vi "Common_UpdateAttributes.vi"(1 "ClassPath/LvClassRef":variant, 2 "NewAttributes":string, 3 "ClassInfo":T4[](array[typedef]), 5 "error in (no error)":errorcluster, 6 "Don't Prompt (False)":bool, 7 "Attributes":T1[](array[typedef]), 8 "Stereotype":string, 9 "Ctl-Description":string) -> (15 "CtlPath":path, 18 "Cancel":bool, 19 "error out":errorcluster)   [LabVIEW 2020] (continued)
                      w703 = 21012 items=[".NET Refnum", "Absolute Value", "Access Rights", "ActiveX Container", "Add", "Add Array Elements", "Agitator", "AllSpoll", "And", "And Array Elements", "Append True/False String", "Application Refnum", "Array", "Array 1", "Array Constant", "Array Max & Min", "Array Size", "Array Subset", "Array To Cluster", "Array To Spreadsheet String", "Array of Strings to Path", "Atmospheric Tank", "Atmospheric Tank 1", "Automation Close", "Automation Open", "Automation Refnum", "Avogadro Constant (1/mol)", "Base 10 Logarithm Of e", "Bin", "Bin 1", "Bluetooth Close Connection", "Bluetooth Create Listener", "Bluetooth Discover", "Bluetooth Network Connection Refnum", "Bluetooth Open Connection", "Bluetooth Read", "Bluetooth Wait On Listener", "Bluetooth Write", "Boolean Array To Number", "Boolean To (0,1)", "Build Array", "Build Cluster Array", "Build Path", "Build Waveform", "Bundle", "Bundle By Name", "Byte Array To String", "Byte Stream File Refnum", "Call By Reference Node", "Call Chain", "Call Library Function Node", "Cancel Button", "Cancel Button 1", "Cancel Notification", "Carriage Return Constant", "Case Structure", "Cast Unit Bases", "Check Valve", "Checkbox", "Class Specifier Constant", "Classic Radio Buttons", "Close File", "Close Reference", "Cluster", "Cluster 1", "Cluster Constant", "Cluster To Array", "Code Interface Node", "Color Box", "Color Box Constant", "Color Box Thin Border", "Color Ramp", "Combo Box", "Combo Box 1", "Combo Box Constant", "Complex Conjugate", "Complex To Polar", "Complex To Re/Im", "Compound Arithmetic", "Compressor", "Concatenate Strings", "Conditional Disable Structure", "Constructor Node", "Control Help Window", "Control Online Help", "Control Refnum", "Convert Unit", "Conveyer", "Copy", "Cosecant", "Cosine", "Cotangent", "Create User Event", "Current VI's Menubar", "Current VI's Path", "DAQmx Analog Trigger Source", "DAQmx Analog Trigger Source 1", "DAQmx Analog Trigger Source 2", "DAQmx Analog Trigger Source Constant", "DAQmx Device Name", "DAQmx Device Name 1", "DAQmx Device Name 2", "DAQmx Device Name Constant", "DAQmx Global Channel", "DAQmx Global Channel 1", "DAQmx Global Channel 2", "DAQmx Global Channel Constant", "DAQmx Physical Channel", "DAQmx Physical Channel 1", "DAQmx Physical Channel 2", "DAQmx Physical Channel Constant", "DAQmx Scale Name", "DAQmx Scale Name 1", "DAQmx Scale Name 2", "DAQmx Scale Name Constant", "DAQmx Switch", "DAQmx Switch 1", "DAQmx Switch 2", "DAQmx Switch Constant", "DAQmx Task Name", "DAQmx Task Name 1", "DAQmx Task Name 2", "DAQmx Task Name Constant", "DAQmx Terminal", "DAQmx Terminal 1", "DAQmx Terminal 2", "DAQmx Terminal Constant", "Data Log File Refnum", "DataSocket Close", "DataSocket Open", "DataSocket Read", "DataSocket Refnum", "DataSocket Write", "Database Variant To Data", "Date/Time To Seconds", "Decimal Digit?", "Decimal String To Number", "Decimate 1D Array", "Decrement", "Default Directory", "Delete", "Delete From Array", "Delete Menu Items", "Delete Variant Attribute", "Delete Waveform Attribute", "Dequeue Element", "Destroy User Event", "DevClear", "DevClearList", "Device Control/Status", "Device Refnum", "Diagram Disable Structure", "Dial", "Dial 1", "Dialog Button", "Dialog Checkbox", "Dialog Chiseled Line", "Dialog Colored Rectangle", "Dialog Combo Box", "Dialog Horizontal Pointer Slide", "Dialog Horizontal Progress Bar", "Dialog Horizontal Slide", "Dialog Label", "Dialog Listbox", "Dialog Listbox 1", "Dialog Multicolumn Listbox", "Dialog Multiple Selection Multicolumn Listbox", "Dialog Numeric", "Dialog Path Control", "Dialog Pict Ring", "Dialog Radio Button", "Dialog Radio Buttons", "Dialog Recessed Frame", "Dialog Ring", "Dialog Spin Control", "Dialog String", "Dialog Tab Control", "Dialog Table", "Dialog Tree", "Dialog Vertical Pointer Slide", "Dialog Vertical Progress Bar", "Dialog Vertical Slide", "Digital Data", "Digital Data 1", "Digital Waveform Graph", "Digital Waveform Graph 1", "Digital Waveform Graph 2", "Divide", "Dlg CheckBox", "Dlg Horiz Scrollbar", "Dlg Numeric", "Dlg Numeric 2", "Dlg String", "Dlg Vert Scrollbar", "Down Arrow", "Down Bow Valve", "Down Bow Valve 1", "Down Bow Valve 2", "Down Rect Valve", "Down Rect Valve 1", "Down Rect Valve 2", "Down Tee", "Down Tee 1", "EOF", "Elementary Charge (C)", "Empty Path Constant", "Empty String Constant", "Empty String/Path?", "Enable Menu Tracking", "EnableLocal", "EnableRemote", "End of Line Constant", "Enqueue Element", "Enqueue Element At Opposite End", "Enum", "Enum 1", "Enum Constant", "Equal To 0?", "Equal?", "Error Ring Constant", "Event Callback Refnum", "Event Structure", "Exchanger", "Exclusive Or", "Exponential", "Exponential (Arg) -1", "Expression Node", "False Constant", "Feedback Node", "FieldPoint IO Point", "FieldPoint IO Point 1", "FieldPoint IO Point Constant", "File Dialog", "File Path Control", "File Path Control 1", "File Path Indicator", "File Path Indicator 1", "File/Directory Info", "FindLstn", "FindRQS", "First Call?", "Flat Box", "Flat Circle", "Flat Down Triangle", "Flat Frame", "Flat Left Triangle", "Flat Right Triangle", "Flat Round Button", "Flat Rounded Box", "Flat Sequence Structure", "Flat Square Button", "Flat Up Triangle", "Flatten To String", "Flatten To XML", "Flattened String To Variant", "Flush File", "Flush Queue", "For Loop", "Format Date/Time String", "Format Into File", "Format Into String", "Format Value", "Formula Node", "Fract/Exp String To Number", "Framed Color Box", "Framed Color Box 1", "Free Label", "Furnace", "GPIB Clear", "GPIB Initialization", "GPIB Misc", "GPIB Read", "GPIB Serial Poll", "GPIB Status", "GPIB Trigger", "GPIB Wait", "GPIB Write", "Gauge", "Gauge 1", "Generate Front Panel Activity", "Generate Occurrence", "Generate User Event", "Generic Refnum", "Generic Refnum By Reference Flatten", "Generic Refnum Deep Copy", "Generic Refnum Name", "Generic Refnum Tag", "Generic Refnum Tag By Reference Flatten", "Generic Refnum Tag Flatten", "Get Date/Time In Seconds", "Get Date/Time String", "Get Help Window Status", "Get Menu Item Info", "Get Menu Selection", "Get Menu Short Cut Info", "Get Notifier Status", "Get Queue Status", "Get Variant Attribute", "Get Waveform Attribute", "Get Waveform Components", "Global Variable", "Gravitational Constant (N m2/kg2)", "Greater Or Equal To 0?", "Greater Or Equal?", "Greater Than 0?", "Greater?", "Handle Peek", "Handle Poke", "Hex Digit?", "Hexadecimal String To Number", "HiQ-Script", "Hopper", "Hopper 1", "Horiz Line", "Horiz Pipe", "Horiz Pipe 1", "Horizontal Button Box", "Horizontal Fill Slide", "Horizontal Fill Slide 1", "Horizontal Graduated Bar", "Horizontal Pointer Slide", "Horizontal Pointer Slide 1", "Horizontal Progress Bar", "Horizontal Slide", "Horizontal Slide Switch", "Horizontal Smooth Box", "Horizontal Switch", "Horizontal Tank", "Horizontal Toggle Switch", "Horizontal Toggle Switch 1", "Hyperbolic Cosine", "Hyperbolic Sine", "Hyperbolic Tangent", "IMAQ Session", "IP To String", "IVI Delete Session", "IVI Logical Name", "IVI Logical Name 1", "IVI Logical Name Constant", "IVI New Session", "Implies", "In Range and Coerce", "Increment", "Index & Bundle Cluster Array", "Index Array", "Index String Array", "Initialize Array", "Insert Into Array", "Insert Menu Items", "Intensity Chart", "Intensity Chart 1", "Intensity Graph", "Intensity Graph 1", "Interleave 1D Arrays", "Interpolate 1D Array", "Inverse Cosine", "Inverse Hyperbolic Cosine", "Inverse Hyperbolic Sine", "Inverse Hyperbolic Tangent", "Inverse Sine", "Inverse Tangent", "Inverse Tangent (2 Input)", "Invoke Node", "IrDA Close Connection", "IrDA Create Listener", "IrDA Discover", "IrDA Network Connection Refnum", "IrDA Open Connection", "IrDA Read", "IrDA Wait On Listener", "IrDA Write", "Join Numbers", "Knob", "Knob 1", "LED Button", "Label", "Labeled Oblong Button", "Labeled Rectangular Button", "Labeled Round Button", "Labeled Square Button", "Left Arrow", "Left Bow Valve", "Left Bow Valve 1", "Left Bow Valve 2", "Left Down Elbow", "Left Down Elbow 1", "Left Pump", "Left Pump 1", "Left Rect Valve", "Left Rect Valve 1", "Left Rect Valve 2", "Left Tee", "Left Tee 1", "Left Up Elbow", "Left Up Elbow 1", "Less Or Equal To 0?", "Less Or Equal?", "Less Than 0?", "Less?", "Lexical Class", "Line Feed Constant", "List Directory", "Listbox", "Listbox 1", "Listbox Symbol Ring Constant", "Local Variable", "Lock Range", "Logarithm Base 10", "Logarithm Base 2", "Logarithm Base X", "Logical Shift", "Lowered Rounded Box", "MATLAB Script", "MakeAddr", "Mantissa & Exponent", "Match First String", "Match Pattern", "Match True/False String", "Max & Min", "Menu Refnum", "Menu Ring", "Menu Ring 1", "Menu-Popup Ring", "Merge Signals", "Meter", "Meter 1", "Molar Gas Constant (J/(mol K))", "Motion Resource", "Motion Resource 1", "Motion Resource Constant", "Motor", "Motor 1", "Move", "Multicolumn Listbox", "Multicolumn Listbox 1", "Multicolumn Listbox 2", "Multicolumn Listbox 3", "Multicolumn Listbox 4", "Multiple Selection Listbox", "Multiple Selection Listbox 1", "Multiple Selection Listbox 2", "Multiple Selection Listbox 3", "Multiple Selection Multicolumn Listbox", "Multiply", "Multiply Array Elements", "Natural Logarithm", "Natural Logarithm (Arg +1)", "Natural Logarithm Base", "Natural Logarithm Of 10", "Natural Logarithm Of 2", "Natural Logarithm Of Pi", "Negate", "Negative Infinity", "New Directory", "New File", "New VI", "New VI Object", "Not", "Not A Number/Path/Refnum?", "Not A Path Constant", "Not And", "Not Equal To 0?", "Not Equal?", "Not Exclusive Or", "Not Or", "Not a Refnum Constant", "Not a Tag", "Number To Boolean Array", "Number To Decimal String", "Number To Engineering String", "Number To Exponential String", "Number To Fractional String", "Number To Hexadecimal String", "Number To Octal String", "Numeric Constant", "Numeric Control", "Numeric Control 1", "Numeric Indicator", "Numeric Indicator 1", "OK Button", "OLE Variant", "Obtain Notifier", "Obtain Queue", "Occurrence Refnum", "Octal Digit?", "Octal String To Number", "Old VISA Open", "One Button Dialog", "Open Application Reference", "Open Device", "Open File", "Open File (New)", "Open Tank", "Open Tank 1", "Open VI Object Reference", "Open VI Reference", "Or", "Or Array Elements", "PPoll", "PPollConfig", "PPollUnconfig", "PassControl", "Path Constant", "Path To String", "Path Type", "Path to Array of Strings", "Pi", "Pi Divided By 2", "Pi Multiplied By 2", "Pick Line", "Pict Ring", "Pict Ring 1", "Picture", "PixMap", "PixMap (Do not touch it!!)", "Planck Constant (J/Hz)", "Platform Flat Square Button", "Plug-In Control", "Polar To Complex", "Positive Infinity", "Power Of 10", "Power Of 2", "Power Of X", "Pressure Tank", "Pressure Tank 1", "Preview Queue Element", "Printable?", "Property Node", "Pulldown Menu Ring", "Push Button", "Quit LabVIEW", "Quotient & Remainder", "Radio Buttons", "Raised Box", "Raised Box 1", "Raised Circle", "Raised Down Triangle", "Raised Frame", "Raised Left Triangle", "Raised Right Triangle", "Raised Rounded Box", "Raised Up Triangle", "Random Number (0-1)", "RcvRespMsg", "Re/Im To Complex", "Read Binary File", "Read Device", "Read File", "ReadStatus", "Receive", "ReceiveSetup", "Recessed Box", "Recessed Circle", "Recessed Down Triangle", "Recessed Frame", "Recessed Left Triangle", "Recessed Menu Ring", "Recessed Right Triangle", "Recessed Rounded Box", "Recessed Up Triangle", "Reciprocal", "Reciprocal Of Pi", "Reciprocal Of e", "Rectangular Stop Button", "Refnum to Path", "Refnum to Session", "Register Event Callback", "Register For Events", "Register Session", "Release Notifier", "Release Queue", "Replace Array Subset", "Replace Substring", "Request Deallocation", "ResetSys", "Reshape Array", "Reverse 1D Array", "Reverse String", "Right Arrow", "Right Bow Valve", "Right Bow Valve 1", "Right Bow Valve 2", "Right Down Elbow", "Right Down Elbow 1", "Right Pump", "Right Pump 1", "Right Rect Valve", "Right Rect Valve 1", "Right Rect Valve 2", "Right Tee", "Right Tee 1", "Right Up Elbow", "Right Up Elbow 1", "Ring Constant", "Rocker", "Rotary Feeder", "Rotate", "Rotate 1D Array", "Rotate Left With Carry", "Rotate Right With Carry", "Rotate String", "Round Button", "Round LED", "Round LED 1", "Round Light", "Round Push Button", "Round Push Button 2", "Round Radio Button", "Round Stop Button", "Round To +Infinity", "Round To -Infinity", "Round To Nearest", "Rydberg Constant (/m)", "Scale By Power Of 2", "Scan From File", "Scan From String", "Scan String For Tokens", "Scan Value", "Search 1D Array", "Search and Replace String", "Search/Split String", "Secant", "Seconds To Date/Time", "Seek", "Select", "Send", "Send Notification", "SendCmds", "SendDataBytes", "SendIFC", "SendLLO", "SendList", "SendSetup", "Session to Refnum", "Set Menu Item Info", "Set Occurrence", "Set Variant Attribute", "Set Waveform Attribute", "SetRWLS", "SetTimeOut", "Sign", "Simple Horizontal Slide", "Simple Numeric", "Simple Numeric 1", "Simple String", "Simple Vertical Slide", "Simulation Loop", "Sinc", "Sine", "Sine & Cosine", "Single Selection Listbox", "Size Handle", "Slide Switch", "Sort 1D Array", "Speed Of Light In Vacuum (m/sec)", "Split 1D Array", "Split Button", "Split Number", "Split Signals", "Spreadsheet String To Array", "Square Button", "Square LED", "Square LED 1", "Square Light", "Square Push Button", "Square Push Button 2", "Square Radio Button", "Square Root", "Stacked Sequence Structure", "Standard ListBox", "State Diagram", "Static VI Reference", "Stop", "Stop Button", "String Constant", "String Control", "String Control 1", "String Indicator", "String Indicator 1", "String Length", "String Subset", "String To Byte Array", "String To IP", "String To Path", "String to Tag", "Strip Path", "SubPanel", "SubPanel (Classic)", "Subtract", "Swap Bytes", "Swap Vector Element", "Swap Words", "TCP Close Connection", "TCP Create Listener", "TCP Flattened Read", "TCP Flattened Write", "TCP Flex Read", "TCP Flex Write", "TCP Network Connection Refnum", "TCP Open Connection", "TCP Read", "TCP Wait On Listener", "TCP Write", "Tab Constant", "Tab Control", "Tab Control 1", "Table", "Table 1", "Table 2", "Tag Attribute Ring", "Tag Constant", "Tag Control", "Tag Control 1", "Tag Indicator", "Tag Indicator 1", "Tag to String", "Tangent", "Tank", "Tank 1", "Temporary Directory", "TestSRQ", "TestSys", "Text & Pict Ring", "Text & Pict Ring 1", "Text Button", "Text Ring", "Text Ring 1", "Thermometer", "Thermometer 1", "Thick Chiseled Line", "Thick Line", "Thick Line with Arrow", "Thick Lowered Box", "Thin Chiseled Line", "Thin Line", "Thin Line with Arrow", "Threshold 1D Array", "Tick Count (ms)", "Time Stamp Constant", "Time Stamp Control", "Time Stamp Control 1", "Time Stamp Indicator", "Time Stamp Indicator 1", "Timed Loop", "To Byte Integer", "To Double Precision Complex", "To Double Precision Float", "To Extended Precision Complex", "To Extended Precision Float", "To Long Integer", "To Lower Case", "To More Generic Class", "To More Specific Class", "To OLE Variant", "To Quad Integer", "To Single Precision Complex", "To Single Precision Float", "To Time Stamp", "To Unsigned Byte Integer", "To Unsigned Long Integer", "To Unsigned Quad Integer", "To Unsigned Word Integer", "To Upper Case", "To Variant", "To Word Integer", "Traditional DAQ Channel", "Traditional DAQ Channel 1", "Traditional DAQ Channel Constant", "Transpose 2D Array", "Tree", "Trigger", "TriggerList", "Two Button Dialog", "Type Cast", "Type and Creator", "UDP Close", "UDP Multicast Open", "UDP Network Connection Refnum", "UDP Open", "UDP Read", "UDP Write", "Unbundle", "Unbundle By Name", "Unflatten From String", "Unflatten From XML", "Uniform Dbl Waveform", "Uniform Int16 Waveform", "Unregister For Events", "Unregister Session", "Up Arrow", "Up Bow Valve", "Up Bow Valve 1", "Up Bow Valve 2", "Up Rect Valve", "Up Rect Valve 1", "Up Rect Valve 2", "Up Tee", "Up Tee 1", "User Item", "VI Library", "VI Refnum", "VISA Assert Interrupt Signal", "VISA Assert Trigger", "VISA Assert Utility Signal", "VISA Clear", "VISA Close", "VISA Disable Event", "VISA Discard Events", "VISA Enable Event", "VISA Find Resource", "VISA Flush I/O Buffer", "VISA GPIB Command", "VISA GPIB Control ATN", "VISA GPIB Control REN", "VISA GPIB Pass Control", "VISA GPIB Send IFC", "VISA In 16", "VISA In 32", "VISA In 8", "VISA Lock", "VISA Map Address", "VISA Map Trigger", "VISA Memory Allocation", "VISA Memory Free", "VISA Move", "VISA Move In 16", "VISA Move In 32", "VISA Move In 8", "VISA Move Out 16", "VISA Move Out 32", "VISA Move Out 8", "VISA Open", "VISA Out 16", "VISA Out 32", "VISA Out 8", "VISA Peek 16", "VISA Peek 32", "VISA Peek 8", "VISA Poke 16", "VISA Poke 32", "VISA Poke 8", "VISA Read", "VISA Read STB", "VISA Read To File", "VISA Refnum to Session", "VISA Resource Name", "VISA Resource Name Constant", "VISA Set I/O Buffer Size", "VISA Status Description", "VISA USB Control In", "VISA USB Control Out", "VISA Unlock", "VISA Unmap Address", "VISA Unmap Trigger", "VISA VXI Cmd or Query", "VISA Wait on Event", "VISA Write", "VISA Write From File", "VISA resource name", "Variant", "Variant To Data", "Variant To Flattened String", "Vert Line", "Vert Pipe", "Vert Pipe 1", "Vert Rocker", "Vertical Fill Slide", "Vertical Fill Slide 1", "Vertical Graduated Bar", "Vertical Pointer Slide", "Vertical Pointer Slide 1", "Vertical Progress Bar", "Vertical Slide", "Vertical Slide Switch", "Vertical Slide Switch 1", "Vertical Smooth Box", "Vertical Switch", "Vertical Toggle Switch", "Vertical Toggle Switch 1", "Volume Info", "Wait (ms)", "Wait For Activity", "Wait For Front Panel Activity", "Wait Until Next ms Multiple", "Wait for GPIB RQS", "Wait on Notification", "Wait on Notification from Multiple", "Wait on Occurrence", "WaitSRQ", "Waveform Chart", "Waveform Chart 1", "Waveform Chart 2", "Waveform Graph", "Waveform Graph 1", "While Loop", "While Loop 1", "White Space?", "Write Device", "Write File", "XY Graph", "XY Graph 1", "Xmath Script"]
                      w706 = refnum<vi> refnum  # Cluster
                      w707 = 3400 items=[".NET Refnum", "Absolute Value", "Access Rights", "ActiveX Container", "Add", "Add Array Elements", "Agitator", "AllSpoll", "And", "And Array Elements", "Append True/False String", "Application Refnum", "Array", "Array 1", "Array Constant", "Array Max & Min", "Array Size", "Array Subset", "Array To Cluster", "Array To Spreadsheet String", "Array of Strings to Path", "Atmospheric Tank", "Atmospheric Tank 1", "Automation Close", "Automation Open", "Automation Refnum", "Avogadro Constant (1/mol)", "Base 10 Logarithm Of e", "Bin", "Bin 1", "Bluetooth Close Connection", "Bluetooth Create Listener", "Bluetooth Discover", "Bluetooth Network Connection Refnum", "Bluetooth Open Connection", "Bluetooth Read", "Bluetooth Wait On Listener", "Bluetooth Write", "Boolean Array To Number", "Boolean To (0,1)", "Build Array", "Build Cluster Array", "Build Path", "Build Waveform", "Bundle", "Bundle By Name", "Byte Array To String", "Byte Stream File Refnum", "Call By Reference Node", "Call Chain", "Call Library Function Node", "Cancel Button", "Cancel Button 1", "Cancel Notification", "Carriage Return Constant", "Case Structure", "Cast Unit Bases", "Check Valve", "Checkbox", "Class Specifier Constant", "Classic Radio Buttons", "Close File", "Close Reference", "Cluster", "Cluster 1", "Cluster Constant", "Cluster To Array", "Code Interface Node", "Color Box", "Color Box Constant", "Color Box Thin Border", "Color Ramp", "Combo Box", "Combo Box 1", "Combo Box Constant", "Complex Conjugate", "Complex To Polar", "Complex To Re/Im", "Compound Arithmetic", "Compressor", "Concatenate Strings", "Conditional Disable Structure", "Constructor Node", "Control Help Window", "Control Online Help", "Control Refnum", "Convert Unit", "Conveyer", "Copy", "Cosecant", "Cosine", "Cotangent", "Create User Event", "Current VI's Menubar", "Current VI's Path", "DAQmx Analog Trigger Source", "DAQmx Analog Trigger Source 1", "DAQmx Analog Trigger Source 2", "DAQmx Analog Trigger Source Constant", "DAQmx Device Name", "DAQmx Device Name 1", "DAQmx Device Name 2", "DAQmx Device Name Constant", "DAQmx Global Channel", "DAQmx Global Channel 1", "DAQmx Global Channel 2", "DAQmx Global Channel Constant", "DAQmx Physical Channel", "DAQmx Physical Channel 1", "DAQmx Physical Channel 2", "DAQmx Physical Channel Constant", "DAQmx Scale Name", "DAQmx Scale Name 1", "DAQmx Scale Name 2", "DAQmx Scale Name Constant", "DAQmx Switch", "DAQmx Switch 1", "DAQmx Switch 2", "DAQmx Switch Constant", "DAQmx Task Name", "DAQmx Task Name 1", "DAQmx Task Name 2", "DAQmx Task Name Constant", "DAQmx Terminal", "DAQmx Terminal 1", "DAQmx Terminal 2", "DAQmx Terminal Constant", "Data Log File Refnum", "DataSocket Close", "DataSocket Open", "DataSocket Read", "DataSocket Refnum", "DataSocket Write", "Database Variant To Data", "Date/Time To Seconds", "Decimal Digit?", "Decimal String To Number", "Decimate 1D Array", "Decrement", "Default Directory", "Delete", "Delete From Array", "Delete Menu Items", "Delete Variant Attribute", "Delete Waveform Attribute", "Dequeue Element", "Destroy User Event", "DevClear", "DevClearList", "Device Control/Status", "Device Refnum", "Diagram Disable Structure", "Dial", "Dial 1", "Dialog Button", "Dialog Checkbox", "Dialog Chiseled Line", "Dialog Colored Rectangle", "Dialog Combo Box", "Dialog Horizontal Pointer Slide", "Dialog Horizontal Progress Bar", "Dialog Horizontal Slide", "Dialog Label", "Dialog Listbox", "Dialog Listbox 1", "Dialog Multicolumn Listbox", "Dialog Multiple Selection Multicolumn Listbox", "Dialog Numeric", "Dialog Path Control", "Dialog Pict Ring", "Dialog Radio Button", "Dialog Radio Buttons", "Dialog Recessed Frame", "Dialog Ring", "Dialog Spin Control", "Dialog String", "Dialog Tab Control", "Dialog Table", "Dialog Tree", "Dialog Vertical Pointer Slide", "Dialog Vertical Progress Bar", "Dialog Vertical Slide", "Digital Data", "Digital Data 1", "Digital Waveform Graph", "Digital Waveform Graph 1", "Digital Waveform Graph 2", "Divide", "Dlg CheckBox", "Dlg Horiz Scrollbar", "Dlg Numeric", "Dlg Numeric 2", "Dlg String", "Dlg Vert Scrollbar", "Down Arrow", "Down Bow Valve", "Down Bow Valve 1", "Down Bow Valve 2", "Down Rect Valve", "Down Rect Valve 1", "Down Rect Valve 2", "Down Tee", "Down Tee 1", "EOF", "Elementary Charge (C)", "Empty Path Constant", "Empty String Constant", "Empty String/Path?", "Enable Menu Tracking", "EnableLocal", "EnableRemote", "End of Line Constant", "Enqueue Element", "Enqueue Element At Opposite End", "Enum", "Enum 1", "Enum Constant", "Equal To 0?", "Equal?", "Error Ring Constant", "Event Callback Refnum", "Event Structure", "Exchanger", "Exclusive Or", "Exponential", "Exponential (Arg) -1", "Expression Node", "False Constant", "Feedback Node", "FieldPoint IO Point", "FieldPoint IO Point 1", "FieldPoint IO Point Constant", "File Dialog", "File Path Control", "File Path Control 1", "File Path Indicator", "File Path Indicator 1", "File/Directory Info", "FindLstn", "FindRQS", "First Call?", "Flat Box", "Flat Circle", "Flat Down Triangle", "Flat Frame", "Flat Left Triangle", "Flat Right Triangle", "Flat Round Button", "Flat Rounded Box", "Flat Sequence Structure", "Flat Square Button", "Flat Up Triangle", "Flatten To String", "Flatten To XML", "Flattened String To Variant", "Flush File", "Flush Queue", "For Loop", "Format Date/Time String", "Format Into File", "Format Into String", "Format Value", "Formula Node", "Fract/Exp String To Number", "Framed Color Box", "Framed Color Box 1", "Free Label", "Furnace", "GPIB Clear", "GPIB Initialization", "GPIB Misc", "GPIB Read", "GPIB Serial Poll", "GPIB Status", "GPIB Trigger", "GPIB Wait", "GPIB Write", "Gauge", "Gauge 1", "Generate Front Panel Activity", "Generate Occurrence", "Generate User Event", "Generic Refnum", "Generic Refnum By Reference Flatten", "Generic Refnum Deep Copy", "Generic Refnum Name", "Generic Refnum Tag", "Generic Refnum Tag By Reference Flatten", "Generic Refnum Tag Flatten", "Get Date/Time In Seconds", "Get Date/Time String", "Get Help Window Status", "Get Menu Item Info", "Get Menu Selection", "Get Menu Short Cut Info", "Get Notifier Status", "Get Queue Status", "Get Variant Attribute", "Get Waveform Attribute", "Get Waveform Components", "Global Variable", "Gravitational Constant (N m2/kg2)", "Greater Or Equal To 0?", "Greater Or Equal?", "Greater Than 0?", "Greater?", "Handle Peek", "Handle Poke", "Hex Digit?", "Hexadecimal String To Number", "HiQ-Script", "Hopper", "Hopper 1", "Horiz Line", "Horiz Pipe", "Horiz Pipe 1", "Horizontal Button Box", "Horizontal Fill Slide", "Horizontal Fill Slide 1", "Horizontal Graduated Bar", "Horizontal Pointer Slide", "Horizontal Pointer Slide 1", "Horizontal Progress Bar", "Horizontal Slide", "Horizontal Slide Switch", "Horizontal Smooth Box", "Horizontal Switch", "Horizontal Tank", "Horizontal Toggle Switch", "Horizontal Toggle Switch 1", "Hyperbolic Cosine", "Hyperbolic Sine", "Hyperbolic Tangent", "IMAQ Session", "IP To String", "IVI Delete Session", "IVI Logical Name", "IVI Logical Name 1", "IVI Logical Name Constant", "IVI New Session", "Implies", "In Range and Coerce", "Increment", "Index & Bundle Cluster Array", "Index Array", "Index String Array", "Initialize Array", "Insert Into Array", "Insert Menu Items", "Intensity Chart", "Intensity Chart 1", "Intensity Graph", "Intensity Graph 1", "Interleave 1D Arrays", "Interpolate 1D Array", "Inverse Cosine", "Inverse Hyperbolic Cosine", "Inverse Hyperbolic Sine", "Inverse Hyperbolic Tangent", "Inverse Sine", "Inverse Tangent", "Inverse Tangent (2 Input)", "Invoke Node", "IrDA Close Connection", "IrDA Create Listener", "IrDA Discover", "IrDA Network Connection Refnum", "IrDA Open Connection", "IrDA Read", "IrDA Wait On Listener", "IrDA Write", "Join Numbers", "Knob", "Knob 1", "LED Button", "Label", "Labeled Oblong Button", "Labeled Rectangular Button", "Labeled Round Button", "Labeled Square Button", "Left Arrow", "Left Bow Valve", "Left Bow Valve 1", "Left Bow Valve 2", "Left Down Elbow", "Left Down Elbow 1", "Left Pump", "Left Pump 1", "Left Rect Valve", "Left Rect Valve 1", "Left Rect Valve 2", "Left Tee", "Left Tee 1", "Left Up Elbow", "Left Up Elbow 1", "Less Or Equal To 0?", "Less Or Equal?", "Less Than 0?", "Less?", "Lexical Class", "Line Feed Constant", "List Directory", "Listbox", "Listbox 1", "Listbox Symbol Ring Constant", "Local Variable", "Lock Range", "Logarithm Base 10", "Logarithm Base 2", "Logarithm Base X", "Logical Shift", "Lowered Rounded Box", "MATLAB Script", "MakeAddr", "Mantissa & Exponent", "Match First String", "Match Pattern", "Match True/False String", "Max & Min", "Menu Refnum", "Menu Ring", "Menu Ring 1", "Menu-Popup Ring", "Merge Signals", "Meter", "Meter 1", "Molar Gas Constant (J/(mol K))", "Motion Resource", "Motion Resource 1", "Motion Resource Constant", "Motor", "Motor 1", "Move", "Multicolumn Listbox", "Multicolumn Listbox 1", "Multicolumn Listbox 2", "Multicolumn Listbox 3", "Multicolumn Listbox 4", "Multiple Selection Listbox", "Multiple Selection Listbox 1", "Multiple Selection Listbox 2", "Multiple Selection Listbox 3", "Multiple Selection Multicolumn Listbox", "Multiply", "Multiply Array Elements", "Natural Logarithm", "Natural Logarithm (Arg +1)", "Natural Logarithm Base", "Natural Logarithm Of 10", "Natural Logarithm Of 2", "Natural Logarithm Of Pi", "Negate", "Negative Infinity", "New Directory", "New File", "New VI", "New VI Object", "Not", "Not A Number/Path/Refnum?", "Not A Path Constant", "Not And", "Not Equal To 0?", "Not Equal?", "Not Exclusive Or", "Not Or", "Not a Refnum Constant", "Not a Tag", "Number To Boolean Array", "Number To Decimal String", "Number To Engineering String", "Number To Exponential String", "Number To Fractional String", "Number To Hexadecimal String", "Number To Octal String", "Numeric Constant", "Numeric Control", "Numeric Control 1", "Numeric Indicator", "Numeric Indicator 1", "OK Button", "OLE Variant", "Obtain Notifier", "Obtain Queue", "Occurrence Refnum", "Octal Digit?", "Octal String To Number", "Old VISA Open", "One Button Dialog", "Open Application Reference", "Open Device", "Open File", "Open File (New)", "Open Tank", "Open Tank 1", "Open VI Object Reference", "Open VI Reference", "Or", "Or Array Elements", "PPoll", "PPollConfig", "PPollUnconfig", "PassControl", "Path Constant", "Path To String", "Path Type", "Path to Array of Strings", "Pi", "Pi Divided By 2", "Pi Multiplied By 2", "Pick Line", "Pict Ring", "Pict Ring 1", "Picture", "PixMap", "PixMap (Do not touch it!!)", "Planck Constant (J/Hz)", "Platform Flat Square Button", "Plug-In Control", "Polar To Complex", "Positive Infinity", "Power Of 10", "Power Of 2", "Power Of X", "Pressure Tank", "Pressure Tank 1", "Preview Queue Element", "Printable?", "Property Node", "Pulldown Menu Ring", "Push Button", "Quit LabVIEW", "Quotient & Remainder", "Radio Buttons", "Raised Box", "Raised Box 1", "Raised Circle", "Raised Down Triangle", "Raised Frame", "Raised Left Triangle", "Raised Right Triangle", "Raised Rounded Box", "Raised Up Triangle", "Random Number (0-1)", "RcvRespMsg", "Re/Im To Complex", "Read Binary File", "Read Device", "Read File", "ReadStatus", "Receive", "ReceiveSetup", "Recessed Box", "Recessed Circle", "Recessed Down Triangle", "Recessed Frame", "Recessed Left Triangle", "Recessed Menu Ring", "Recessed Right Triangle", "Recessed Rounded Box", "Recessed Up Triangle", "Reciprocal", "Reciprocal Of Pi", "Reciprocal Of e", "Rectangular Stop Button", "Refnum to Path", "Refnum to Session", "Register Event Callback", "Register For Events", "Register Session", "Release Notifier", "Release Queue", "Replace Array Subset", "Replace Substring", "Request Deallocation", "ResetSys", "Reshape Array", "Reverse 1D Array", "Reverse String", "Right Arrow", "Right Bow Valve", "Right Bow Valve 1", "Right Bow Valve 2", "Right Down Elbow", "Right Down Elbow 1", "Right Pump", "Right Pump 1", "Right Rect Valve", "Right Rect Valve 1", "Right Rect Valve 2", "Right Tee", "Right Tee 1", "Right Up Elbow", "Right Up Elbow 1", "Ring Constant", "Rocker", "Rotary Feeder", "Rotate", "Rotate 1D Array", "Rotate Left With Carry", "Rotate Right With Carry", "Rotate String", "Round Button", "Round LED", "Round LED 1", "Round Light", "Round Push Button", "Round Push Button 2", "Round Radio Button", "Round Stop Button", "Round To +Infinity", "Round To -Infinity", "Round To Nearest", "Rydberg Constant (/m)", "Scale By Power Of 2", "Scan From File", "Scan From String", "Scan String For Tokens", "Scan Value", "Search 1D Array", "Search and Replace String", "Search/Split String", "Secant", "Seconds To Date/Time", "Seek", "Select", "Send", "Send Notification", "SendCmds", "SendDataBytes", "SendIFC", "SendLLO", "SendList", "SendSetup", "Session to Refnum", "Set Menu Item Info", "Set Occurrence", "Set Variant Attribute", "Set Waveform Attribute", "SetRWLS", "SetTimeOut", "Sign", "Simple Horizontal Slide", "Simple Numeric", "Simple Numeric 1", "Simple String", "Simple Vertical Slide", "Simulation Loop", "Sinc", "Sine", "Sine & Cosine", "Single Selection Listbox", "Size Handle", "Slide Switch", "Sort 1D Array", "Speed Of Light In Vacuum (m/sec)", "Split 1D Array", "Split Button", "Split Number", "Split Signals", "Spreadsheet String To Array", "Square Button", "Square LED", "Square LED 1", "Square Light", "Square Push Button", "Square Push Button 2", "Square Radio Button", "Square Root", "Stacked Sequence Structure", "Standard ListBox", "State Diagram", "Static VI Reference", "Stop", "Stop Button", "String Constant", "String Control", "String Control 1", "String Indicator", "String Indicator 1", "String Length", "String Subset", "String To Byte Array", "String To IP", "String To Path", "String to Tag", "Strip Path", "SubPanel", "SubPanel (Classic)", "Subtract", "Swap Bytes", "Swap Vector Element", "Swap Words", "TCP Close Connection", "TCP Create Listener", "TCP Flattened Read", "TCP Flattened Write", "TCP Flex Read", "TCP Flex Write", "TCP Network Connection Refnum", "TCP Open Connection", "TCP Read", "TCP Wait On Listener", "TCP Write", "Tab Constant", "Tab Control", "Tab Control 1", "Table", "Table 1", "Table 2", "Tag Attribute Ring", "Tag Constant", "Tag Control", "Tag Control 1", "Tag Indicator", "Tag Indicator 1", "Tag to String", "Tangent", "Tank", "Tank 1", "Temporary Directory", "TestSRQ", "TestSys", "Text & Pict Ring", "Text & Pict Ring 1", "Text Button", "Text Ring", "Text Ring 1", "Thermometer", "Thermometer 1", "Thick Chiseled Line", "Thick Line", "Thick Line with Arrow", "Thick Lowered Box", "Thin Chiseled Line", "Thin Line", "Thin Line with Arrow", "Threshold 1D Array", "Tick Count (ms)", "Time Stamp Constant", "Time Stamp Control", "Time Stamp Control 1", "Time Stamp Indicator", "Time Stamp Indicator 1", "Timed Loop", "To Byte Integer", "To Double Precision Complex", "To Double Precision Float", "To Extended Precision Complex", "To Extended Precision Float", "To Long Integer", "To Lower Case", "To More Generic Class", "To More Specific Class", "To OLE Variant", "To Quad Integer", "To Single Precision Complex", "To Single Precision Float", "To Time Stamp", "To Unsigned Byte Integer", "To Unsigned Long Integer", "To Unsigned Quad Integer", "To Unsigned Word Integer", "To Upper Case", "To Variant", "To Word Integer", "Traditional DAQ Channel", "Traditional DAQ Channel 1", "Traditional DAQ Channel Constant", "Transpose 2D Array", "Tree", "Trigger", "TriggerList", "Two Button Dialog", "Type Cast", "Type and Creator", "UDP Close", "UDP Multicast Open", "UDP Network Connection Refnum", "UDP Open", "UDP Read", "UDP Write", "Unbundle", "Unbundle By Name", "Unflatten From String", "Unflatten From XML", "Uniform Dbl Waveform", "Uniform Int16 Waveform", "Unregister For Events", "Unregister Session", "Up Arrow", "Up Bow Valve", "Up Bow Valve 1", "Up Bow Valve 2", "Up Rect Valve", "Up Rect Valve 1", "Up Rect Valve 2", "Up Tee", "Up Tee 1", "User Item", "VI Library", "VI Refnum", "VISA Assert Interrupt Signal", "VISA Assert Trigger", "VISA Assert Utility Signal", "VISA Clear", "VISA Close", "VISA Disable Event", "VISA Discard Events", "VISA Enable Event", "VISA Find Resource", "VISA Flush I/O Buffer", "VISA GPIB Command", "VISA GPIB Control ATN", "VISA GPIB Control REN", "VISA GPIB Pass Control", "VISA GPIB Send IFC", "VISA In 16", "VISA In 32", "VISA In 8", "VISA Lock", "VISA Map Address", "VISA Map Trigger", "VISA Memory Allocation", "VISA Memory Free", "VISA Move", "VISA Move In 16", "VISA Move In 32", "VISA Move In 8", "VISA Move Out 16", "VISA Move Out 32", "VISA Move Out 8", "VISA Open", "VISA Out 16", "VISA Out 32", "VISA Out 8", "VISA Peek 16", "VISA Peek 32", "VISA Peek 8", "VISA Poke 16", "VISA Poke 32", "VISA Poke 8", "VISA Read", "VISA Read STB", "VISA Read To File", "VISA Refnum to Session", "VISA Resource Name", "VISA Resource Name Constant", "VISA Set I/O Buffer Size", "VISA Status Description", "VISA USB Control In", "VISA USB Control Out", "VISA Unlock", "VISA Unmap Address", "VISA Unmap Trigger", "VISA VXI Cmd or Query", "VISA Wait on Event", "VISA Write", "VISA Write From File", "VISA resource name", "Variant", "Variant To Data", "Variant To Flattened String", "Vert Line", "Vert Pipe", "Vert Pipe 1", "Vert Rocker", "Vertical Fill Slide", "Vertical Fill Slide 1", "Vertical Graduated Bar", "Vertical Pointer Slide", "Vertical Pointer Slide 1", "Vertical Progress Bar", "Vertical Slide", "Vertical Slide Switch", "Vertical Slide Switch 1", "Vertical Smooth Box", "Vertical Switch", "Vertical Toggle Switch", "Vertical Toggle Switch 1", "Volume Info", "Wait (ms)", "Wait For Activity", "Wait For Front Panel Activity", "Wait Until Next ms Multiple", "Wait for GPIB RQS", "Wait on Notification", "Wait on Notification from Multiple", "Wait on Occurrence", "WaitSRQ", "Waveform Chart", "Waveform Chart 1", "Waveform Chart 2", "Waveform Graph", "Waveform Graph 1", "While Loop", "While Loop 1", "White Space?", "Write Device", "Write File", "XY Graph", "XY Graph 1", "Xmath Script"]
                      n246 = New VI Object(vi object class=w706, owner refnum=w705, style=w707, position/next to=w704, 4:cluster{"Width":u32, "Height":u32} {"Width"=50, "Height"=50} ("bounds"), 8:w711) -> (object refnum=w697:refnum<vi>, 0:w710:errorcluster)  [unwired: 2 out]
                      n247 = New VI Object(vi object class=w702, owner refnum=w697, style=w703, position/next to=cluster{"Horizontal":i16, "Vertical":i16} {"Horizontal"=0, "Vertical"=20}, 8:w710) -> (object refnum=w700:refnum<vi>, 0:w709:errorcluster)  [unwired: 3 out]
                      n248 = property class="Clust"(reference=w697, error in=w709, "Auto Sizing"=u32 3) -> ()  [unwired: 2 out]
                      n249 = Close Reference(reference=w700, error in (no error)=w709) -> (error out=w708:errorcluster)
                    }
                    frame "TypeDef" {
                      w719 = refnum<vi> refnum  # String
                      w723 = refnum<vi> refnum  # Control
                      w720 = 21701 items=[".NET Refnum", "Absolute Value", "Access Rights", "ActiveX Container", "Add", "Add Array Elements", "Agitator", "AllSpoll", "And", "And Array Elements", "Append True/False String", "Application Refnum", "Array", "Array 1", "Array Constant", "Array Max & Min", "Array Size", "Array Subset", "Array To Cluster", "Array To Spreadsheet String", "Array of Strings to Path", "Atmospheric Tank", "Atmospheric Tank 1", "Automation Close", "Automation Open", "Automation Refnum", "Avogadro Constant (1/mol)", "Base 10 Logarithm Of e", "Bin", "Bin 1", "Bluetooth Close Connection", "Bluetooth Create Listener", "Bluetooth Discover", "Bluetooth Network Connection Refnum", "Bluetooth Open Connection", "Bluetooth Read", "Bluetooth Wait On Listener", "Bluetooth Write", "Boolean Array To Number", "Boolean To (0,1)", "Build Array", "Build Cluster Array", "Build Path", "Build Waveform", "Bundle", "Bundle By Name", "Byte Array To String", "Byte Stream File Refnum", "Call By Reference Node", "Call Chain", "Call Library Function Node", "Cancel Button", "Cancel Button 1", "Cancel Notification", "Carriage Return Constant", "Case Structure", "Cast Unit Bases", "Check Valve", "Checkbox", "Class Specifier Constant", "Classic Radio Buttons", "Close File", "Close Reference", "Cluster", "Cluster 1", "Cluster Constant", "Cluster To Array", "Code Interface Node", "Color Box", "Color Box Constant", "Color Box Thin Border", "Color Ramp", "Combo Box", "Combo Box 1", "Combo Box Constant", "Complex Conjugate", "Complex To Polar", "Complex To Re/Im", "Compound Arithmetic", "Compressor", "Concatenate Strings", "Conditional Disable Structure", "Constructor Node", "Control Help Window", "Control Online Help", "Control Refnum", "Convert Unit", "Conveyer", "Copy", "Cosecant", "Cosine", "Cotangent", "Create User Event", "Current VI's Menubar", "Current VI's Path", "DAQmx Analog Trigger Source", "DAQmx Analog Trigger Source 1", "DAQmx Analog Trigger Source 2", "DAQmx Analog Trigger Source Constant", "DAQmx Device Name", "DAQmx Device Name 1", "DAQmx Device Name 2", "DAQmx Device Name Constant", "DAQmx Global Channel", "DAQmx Global Channel 1", "DAQmx Global Channel 2", "DAQmx Global Channel Constant", "DAQmx Physical Channel", "DAQmx Physical Channel 1", "DAQmx Physical Channel 2", "DAQmx Physical Channel Constant", "DAQmx Scale Name", "DAQmx Scale Name 1", "DAQmx Scale Name 2", "DAQmx Scale Name Constant", "DAQmx Switch", "DAQmx Switch 1", "DAQmx Switch 2", "DAQmx Switch Constant", "DAQmx Task Name", "DAQmx Task Name 1", "DAQmx Task Name 2", "DAQmx Task Name Constant", "DAQmx Terminal", "DAQmx Terminal 1", "DAQmx Terminal 2", "DAQmx Terminal Constant", "Data Log File Refnum", "DataSocket Close", "DataSocket Open", "DataSocket Read", "DataSocket Refnum", "DataSocket Write", "Database Variant To Data", "Date/Time To Seconds", "Decimal Digit?", "Decimal String To Number", "Decimate 1D Array", "Decrement", "Default Directory", "Delete", "Delete From Array", "Delete Menu Items", "Delete Variant Attribute", "Delete Waveform Attribute", "Dequeue Element", "Destroy User Event", "DevClear", "DevClearList", "Device Control/Status", "Device Refnum", "Diagram Disable Structure", "Dial", "Dial 1", "Dialog Button", "Dialog Checkbox", "Dialog Chiseled Line", "Dialog Colored Rectangle", "Dialog Combo Box", "Dialog Horizontal Pointer Slide", "Dialog Horizontal Progress Bar", "Dialog Horizontal Slide", "Dialog Label", "Dialog Listbox", "Dialog Listbox 1", "Dialog Multicolumn Listbox", "Dialog Multiple Selection Multicolumn Listbox", "Dialog Numeric", "Dialog Path Control", "Dialog Pict Ring", "Dialog Radio Button", "Dialog Radio Buttons", "Dialog Recessed Frame", "Dialog Ring", "Dialog Spin Control", "Dialog String", "Dialog Tab Control", "Dialog Table", "Dialog Tree", "Dialog Vertical Pointer Slide", "Dialog Vertical Progress Bar", "Dialog Vertical Slide", "Digital Data", "Digital Data 1", "Digital Waveform Graph", "Digital Waveform Graph 1", "Digital Waveform Graph 2", "Divide", "Dlg CheckBox", "Dlg Horiz Scrollbar", "Dlg Numeric", "Dlg Numeric 2", "Dlg String", "Dlg Vert Scrollbar", "Down Arrow", "Down Bow Valve", "Down Bow Valve 1", "Down Bow Valve 2", "Down Rect Valve", "Down Rect Valve 1", "Down Rect Valve 2", "Down Tee", "Down Tee 1", "EOF", "Elementary Charge (C)", "Empty Path Constant", "Empty String Constant", "Empty String/Path?", "Enable Menu Tracking", "EnableLocal", "EnableRemote", "End of Line Constant", "Enqueue Element", "Enqueue Element At Opposite End", "Enum", "Enum 1", "Enum Constant", "Equal To 0?", "Equal?", "Error Ring Constant", "Event Callback Refnum", "Event Structure", "Exchanger", "Exclusive Or", "Exponential", "Exponential (Arg) -1", "Expression Node", "False Constant", "Feedback Node", "FieldPoint IO Point", "FieldPoint IO Point 1", "FieldPoint IO Point Constant", "File Dialog", "File Path Control", "File Path Control 1", "File Path Indicator", "File Path Indicator 1", "File/Directory Info", "FindLstn", "FindRQS", "First Call?", "Flat Box", "Flat Circle", "Flat Down Triangle", "Flat Frame", "Flat Left Triangle", "Flat Right Triangle", "Flat Round Button", "Flat Rounded Box", "Flat Sequence Structure", "Flat Square Button", "Flat Up Triangle", "Flatten To String", "Flatten To XML", "Flattened String To Variant", "Flush File", "Flush Queue", "For Loop", "Format Date/Time String", "Format Into File", "Format Into String", "Format Value", "Formula Node", "Fract/Exp String To Number", "Framed Color Box", "Framed Color Box 1", "Free Label", "Furnace", "GPIB Clear", "GPIB Initialization", "GPIB Misc", "GPIB Read", "GPIB Serial Poll", "GPIB Status", "GPIB Trigger", "GPIB Wait", "GPIB Write", "Gauge", "Gauge 1", "Generate Front Panel Activity", "Generate Occurrence", "Generate User Event", "Generic Refnum", "Generic Refnum By Reference Flatten", "Generic Refnum Deep Copy", "Generic Refnum Name", "Generic Refnum Tag", "Generic Refnum Tag By Reference Flatten", "Generic Refnum Tag Flatten", "Get Date/Time In Seconds", "Get Date/Time String", "Get Help Window Status", "Get Menu Item Info", "Get Menu Selection", "Get Menu Short Cut Info", "Get Notifier Status", "Get Queue Status", "Get Variant Attribute", "Get Waveform Attribute", "Get Waveform Components", "Global Variable", "Gravitational Constant (N m2/kg2)", "Greater Or Equal To 0?", "Greater Or Equal?", "Greater Than 0?", "Greater?", "Handle Peek", "Handle Poke", "Hex Digit?", "Hexadecimal String To Number", "HiQ-Script", "Hopper", "Hopper 1", "Horiz Line", "Horiz Pipe", "Horiz Pipe 1", "Horizontal Button Box", "Horizontal Fill Slide", "Horizontal Fill Slide 1", "Horizontal Graduated Bar", "Horizontal Pointer Slide", "Horizontal Pointer Slide 1", "Horizontal Progress Bar", "Horizontal Slide", "Horizontal Slide Switch", "Horizontal Smooth Box", "Horizontal Switch", "Horizontal Tank", "Horizontal Toggle Switch", "Horizontal Toggle Switch 1", "Hyperbolic Cosine", "Hyperbolic Sine", "Hyperbolic Tangent", "IMAQ Session", "IP To String", "IVI Delete Session", "IVI Logical Name", "IVI Logical Name 1", "IVI Logical Name Constant", "IVI New Session", "Implies", "In Range and Coerce", "Increment", "Index & Bundle Cluster Array", "Index Array", "Index String Array", "Initialize Array", "Insert Into Array", "Insert Menu Items", "Intensity Chart", "Intensity Chart 1", "Intensity Graph", "Intensity Graph 1", "Interleave 1D Arrays", "Interpolate 1D Array", "Inverse Cosine", "Inverse Hyperbolic Cosine", "Inverse Hyperbolic Sine", "Inverse Hyperbolic Tangent", "Inverse Sine", "Inverse Tangent", "Inverse Tangent (2 Input)", "Invoke Node", "IrDA Close Connection", "IrDA Create Listener", "IrDA Discover", "IrDA Network Connection Refnum", "IrDA Open Connection", "IrDA Read", "IrDA Wait On Listener", "IrDA Write", "Join Numbers", "Knob", "Knob 1", "LED Button", "Label", "Labeled Oblong Button", "Labeled Rectangular Button", "Labeled Round Button", "Labeled Square Button", "Left Arrow", "Left Bow Valve", "Left Bow Valve 1", "Left Bow Valve 2", "Left Down Elbow", "Left Down Elbow 1", "Left Pump", "Left Pump 1", "Left Rect Valve", "Left Rect Valve 1", "Left Rect Valve 2", "Left Tee", "Left Tee 1", "Left Up Elbow", "Left Up Elbow 1", "Less Or Equal To 0?", "Less Or Equal?", "Less Than 0?", "Less?", "Lexical Class", "Line Feed Constant", "List Directory", "Listbox", "Listbox 1", "Listbox Symbol Ring Constant", "Local Variable", "Lock Range", "Logarithm Base 10", "Logarithm Base 2", "Logarithm Base X", "Logical Shift", "Lowered Rounded Box", "MATLAB Script", "MakeAddr", "Mantissa & Exponent", "Match First String", "Match Pattern", "Match True/False String", "Max & Min", "Menu Refnum", "Menu Ring", "Menu Ring 1", "Menu-Popup Ring", "Merge Signals", "Meter", "Meter 1", "Molar Gas Constant (J/(mol K))", "Motion Resource", "Motion Resource 1", "Motion Resource Constant", "Motor", "Motor 1", "Move", "Multicolumn Listbox", "Multicolumn Listbox 1", "Multicolumn Listbox 2", "Multicolumn Listbox 3", "Multicolumn Listbox 4", "Multiple Selection Listbox", "Multiple Selection Listbox 1", "Multiple Selection Listbox 2", "Multiple Selection Listbox 3", "Multiple Selection Multicolumn Listbox", "Multiply", "Multiply Array Elements", "Natural Logarithm", "Natural Logarithm (Arg +1)", "Natural Logarithm Base", "Natural Logarithm Of 10", "Natural Logarithm Of 2", "Natural Logarithm Of Pi", "Negate", "Negative Infinity", "New Directory", "New File", "New VI", "New VI Object", "Not", "Not A Number/Path/Refnum?", "Not A Path Constant", "Not And", "Not Equal To 0?", "Not Equal?", "Not Exclusive Or", "Not Or", "Not a Refnum Constant", "Not a Tag", "Number To Boolean Array", "Number To Decimal String", "Number To Engineering String", "Number To Exponential String", "Number To Fractional String", "Number To Hexadecimal String", "Number To Octal String", "Numeric Constant", "Numeric Control", "Numeric Control 1", "Numeric Indicator", "Numeric Indicator 1", "OK Button", "OLE Variant", "Obtain Notifier", "Obtain Queue", "Occurrence Refnum", "Octal Digit?", "Octal String To Number", "Old VISA Open", "One Button Dialog", "Open Application Reference", "Open Device", "Open File", "Open File (New)", "Open Tank", "Open Tank 1", "Open VI Object Reference", "Open VI Reference", "Or", "Or Array Elements", "PPoll", "PPollConfig", "PPollUnconfig", "PassControl", "Path Constant", "Path To String", "Path Type", "Path to Array of Strings", "Pi", "Pi Divided By 2", "Pi Multiplied By 2", "Pick Line", "Pict Ring", "Pict Ring 1", "Picture", "PixMap", "PixMap (Do not touch it!!)", "Planck Constant (J/Hz)", "Platform Flat Square Button", "Plug-In Control", "Polar To Complex", "Positive Infinity", "Power Of 10", "Power Of 2", "Power Of X", "Pressure Tank", "Pressure Tank 1", "Preview Queue Element", "Printable?", "Property Node", "Pulldown Menu Ring", "Push Button", "Quit LabVIEW", "Quotient & Remainder", "Radio Buttons", "Raised Box", "Raised Box 1", "Raised Circle", "Raised Down Triangle", "Raised Frame", "Raised Left Triangle", "Raised Right Triangle", "Raised Rounded Box", "Raised Up Triangle", "Random Number (0-1)", "RcvRespMsg", "Re/Im To Complex", "Read Binary File", "Read Device", "Read File", "ReadStatus", "Receive", "ReceiveSetup", "Recessed Box", "Recessed Circle", "Recessed Down Triangle", "Recessed Frame", "Recessed Left Triangle", "Recessed Menu Ring", "Recessed Right Triangle", "Recessed Rounded Box", "Recessed Up Triangle", "Reciprocal", "Reciprocal Of Pi", "Reciprocal Of e", "Rectangular Stop Button", "Refnum to Path", "Refnum to Session", "Register Event Callback", "Register For Events", "Register Session", "Release Notifier", "Release Queue", "Replace Array Subset", "Replace Substring", "Request Deallocation", "ResetSys", "Reshape Array", "Reverse 1D Array", "Reverse String", "Right Arrow", "Right Bow Valve", "Right Bow Valve 1", "Right Bow Valve 2", "Right Down Elbow", "Right Down Elbow 1", "Right Pump", "Right Pump 1", "Right Rect Valve", "Right Rect Valve 1", "Right Rect Valve 2", "Right Tee", "Right Tee 1", "Right Up Elbow", "Right Up Elbow 1", "Ring Constant", "Rocker", "Rotary Feeder", "Rotate", "Rotate 1D Array", "Rotate Left With Carry", "Rotate Right With Carry", "Rotate String", "Round Button", "Round LED", "Round LED 1", "Round Light", "Round Push Button", "Round Push Button 2", "Round Radio Button", "Round Stop Button", "Round To +Infinity", "Round To -Infinity", "Round To Nearest", "Rydberg Constant (/m)", "Scale By Power Of 2", "Scan From File", "Scan From String", "Scan String For Tokens", "Scan Value", "Search 1D Array", "Search and Replace String", "Search/Split String", "Secant", "Seconds To Date/Time", "Seek", "Select", "Send", "Send Notification", "SendCmds", "SendDataBytes", "SendIFC", "SendLLO", "SendList", "SendSetup", "Session to Refnum", "Set Menu Item Info", "Set Occurrence", "Set Variant Attribute", "Set Waveform Attribute", "SetRWLS", "SetTimeOut", "Sign", "Simple Horizontal Slide", "Simple Numeric", "Simple Numeric 1", "Simple String", "Simple Vertical Slide", "Simulation Loop", "Sinc", "Sine", "Sine & Cosine", "Single Selection Listbox", "Size Handle", "Slide Switch", "Sort 1D Array", "Speed Of Light In Vacuum (m/sec)", "Split 1D Array", "Split Button", "Split Number", "Split Signals", "Spreadsheet String To Array", "Square Button", "Square LED", "Square LED 1", "Square Light", "Square Push Button", "Square Push Button 2", "Square Radio Button", "Square Root", "Stacked Sequence Structure", "Standard ListBox", "State Diagram", "Static VI Reference", "Stop", "Stop Button", "String Constant", "String Control", "String Control 1", "String Indicator", "String Indicator 1", "String Length", "String Subset", "String To Byte Array", "String To IP", "String To Path", "String to Tag", "Strip Path", "SubPanel", "SubPanel (Classic)", "Subtract", "Swap Bytes", "Swap Vector Element", "Swap Words", "TCP Close Connection", "TCP Create Listener", "TCP Flattened Read", "TCP Flattened Write", "TCP Flex Read", "TCP Flex Write", "TCP Network Connection Refnum", "TCP Open Connection", "TCP Read", "TCP Wait On Listener", "TCP Write", "Tab Constant", "Tab Control", "Tab Control 1", "Table", "Table 1", "Table 2", "Tag Attribute Ring", "Tag Constant", "Tag Control", "Tag Control 1", "Tag Indicator", "Tag Indicator 1", "Tag to String", "Tangent", "Tank", "Tank 1", "Temporary Directory", "TestSRQ", "TestSys", "Text & Pict Ring", "Text & Pict Ring 1", "Text Button", "Text Ring", "Text Ring 1", "Thermometer", "Thermometer 1", "Thick Chiseled Line", "Thick Line", "Thick Line with Arrow", "Thick Lowered Box", "Thin Chiseled Line", "Thin Line", "Thin Line with Arrow", "Threshold 1D Array", "Tick Count (ms)", "Time Stamp Constant", "Time Stamp Control", "Time Stamp Control 1", "Time Stamp Indicator", "Time Stamp Indicator 1", "Timed Loop", "To Byte Integer", "To Double Precision Complex", "To Double Precision Float", "To Extended Precision Complex", "To Extended Precision Float", "To Long Integer", "To Lower Case", "To More Generic Class", "To More Specific Class", "To OLE Variant", "To Quad Integer", "To Single Precision Complex", "To Single Precision Float", "To Time Stamp", "To Unsigned Byte Integer", "To Unsigned Long Integer", "To Unsigned Quad Integer", "To Unsigned Word Integer", "To Upper Case", "To Variant", "To Word Integer", "Traditional DAQ Channel", "Traditional DAQ Channel 1", "Traditional DAQ Channel Constant", "Transpose 2D Array", "Tree", "Trigger", "TriggerList", "Two Button Dialog", "Type Cast", "Type and Creator", "UDP Close", "UDP Multicast Open", "UDP Network Connection Refnum", "UDP Open", "UDP Read", "UDP Write", "Unbundle", "Unbundle By Name", "Unflatten From String", "Unflatten From XML", "Uniform Dbl Waveform", "Uniform Int16 Waveform", "Unregister For Events", "Unregister Session", "Up Arrow", "Up Bow Valve", "Up Bow Valve 1", "Up Bow Valve 2", "Up Rect Valve", "Up Rect Valve 1", "Up Rect Valve 2", "Up Tee", "Up Tee 1", "User Item", "VI Library", "VI Refnum", "VISA Assert Interrupt Signal", "VISA Assert Trigger", "VISA Assert Utility Signal", "VISA Clear", "VISA Close", "VISA Disable Event", "VISA Discard Events", "VISA Enable Event", "VISA Find Resource", "VISA Flush I/O Buffer", "VISA GPIB Command", "VISA GPIB Control ATN", "VISA GPIB Control REN", "VISA GPIB Pass Control", "VISA GPIB Send IFC", "VISA In 16", "VISA In 32", "VISA In 8", "VISA Lock", "VISA Map Address", "VISA Map Trigger", "VISA Memory Allocation", "VISA Memory Free", "VISA Move", "VISA Move In 16", "VISA Move In 32", "VISA Move In 8", "VISA Move Out 16", "VISA Move Out 32", "VISA Move Out 8", "VISA Open", "VISA Out 16", "VISA Out 32", "VISA Out 8", "VISA Peek 16", "VISA Peek 32", "VISA Peek 8", "VISA Poke 16", "VISA Poke 32", "VISA Poke 8", "VISA Read", "VISA Read STB", "VISA Read To File", "VISA Refnum to Session", "VISA Resource Name", "VISA Resource Name Constant", "VISA Set I/O Buffer Size", "VISA Status Description", "VISA USB Control In", "VISA USB Control Out", "VISA Unlock", "VISA Unmap Address", "VISA Unmap Trigger", "VISA VXI Cmd or Query", "VISA Wait on Event", "VISA Write", "VISA Write From File", "VISA resource name", "Variant", "Variant To Data", "Variant To Flattened String", "Vert Line", "Vert Pipe", "Vert Pipe 1", "Vert Rocker", "Vertical Fill Slide", "Vertical Fill Slide 1", "Vertical Graduated Bar", "Vertical Pointer Slide", "Vertical Pointer Slide 1", "Vertical Progress Bar", "Vertical Slide", "Vertical Slide Switch", "Vertical Slide Switch 1", "Vertical Smooth Box", "Vertical Switch", "Vertical Toggle Switch", "Vertical Toggle Switch 1", "Volume Info", "Wait (ms)", "Wait For Activity", "Wait For Front Panel Activity", "Wait Until Next ms Multiple", "Wait for GPIB RQS", "Wait on Notification", "Wait on Notification from Multiple", "Wait on Occurrence", "WaitSRQ", "Waveform Chart", "Waveform Chart 1", "Waveform Chart 2", "Waveform Graph", "Waveform Graph 1", "While Loop", "While Loop 1", "White Space?", "Write Device", "Write File", "XY Graph", "XY Graph 1", "Xmath Script"]
                      n250 = call "Common_TempCangeLabelName.vi"("Path"=w715, "String"=w713) -> ("PathOut"=w714:path)  [unwired: 17 out]
                      n251 = New VI Object(vi object class=w723, owner refnum=w717, position/next to=w718, 6:w714, 8:w725) -> (object refnum=w716:refnum<vi>, 0:w724:errorcluster)  [unwired: 1 in, 2 out]
                      n252 = Unbundle By Name(w724) -> ("code"=w722:i32)
                      n253 = case shown="1059, 1061" w722 {
                        tunnel: w724 -> [w729 _]
                        tunnel: [w729 w737] -> w726
                        tunnel: w716 -> [w728 _]
                        tunnel: [w728 w733] -> w721
                        tunnel: w720 -> [_ w735]
                        tunnel: w719 -> [_ w734]
                        tunnel: w718 -> [_ w731]
                        tunnel: w717 -> [_ w730]
                        tunnel: w725 -> [_ w736]
                        tunnel: ["" _] -> w712
                        frame Default {
                        }
                        frame 1059, 1061 {
                          n254 = New VI Object(vi object class=w734, owner refnum=w730, style=w735, position/next to=w731, 8:w736) -> (object refnum=w733:refnum<vi>, 0:w737:errorcluster)  [unwired: 3 out]
                          n255 = One Button Dialog(message="WARNING\nCould not find the type-def file to create, or the type-def is broken.\n\nThe LabVIEW scripting, don't support type-def that are \"Brooken\" or \"Not OK\".\nMake sure the type-defs are ok before doing this again.") -> ()  [unwired: 2 out]
                        }
                      }
                      n256 = call "Common_TempCangeLabelName.vi"("String"=w712) -> ()  [unwired: 1 in, 18 out]
                    }
                    frame "VIRefNum" {
                      w741 = refnum<vi> refnum  # VIRefNum
